vi "Check MCP Names.vi"(8 "error in":errorcluster, 9 "kind (Control)":string="Control", 10 "labels":string[](array[string]), 11 "MCP names":string[](array[string])) -> (0 "error out":errorcluster)   [LabVIEW 2020, in "MCP Server.lvlib"]
doc: "Checks MCP names generated by To MCP Name.vi before a tool or prompt is registered. Returns error 5010 when a name is empty, when it is longer than 64 characters, or when two different labels map to the same MCP name. The error message names the offending label(s) and the generated name. Passes an incoming error through unchanged."
uses:
  MCP Server.lvlib
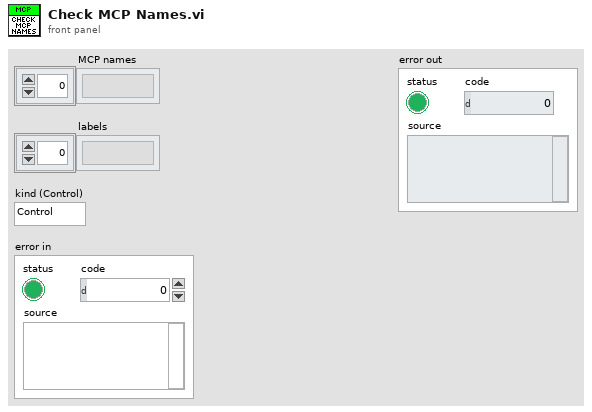
[diagram p1: front panel]
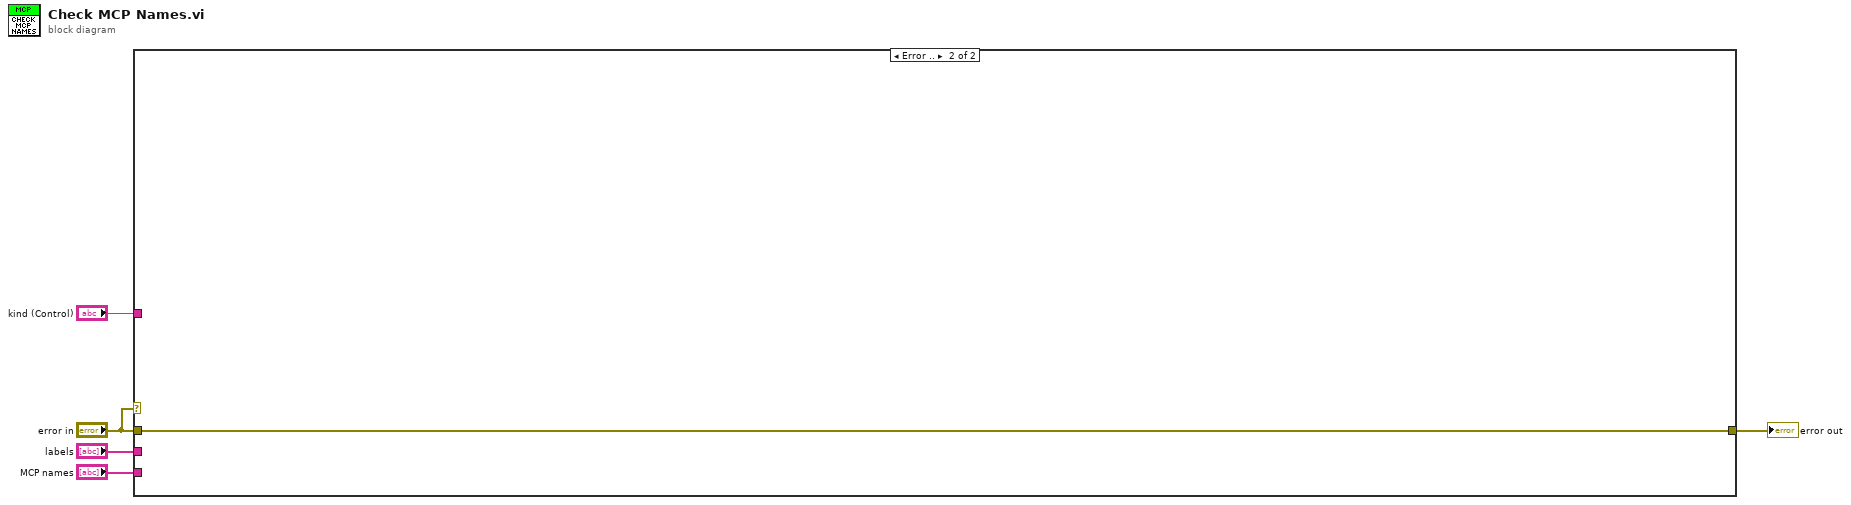
[diagram p0: block diagram]
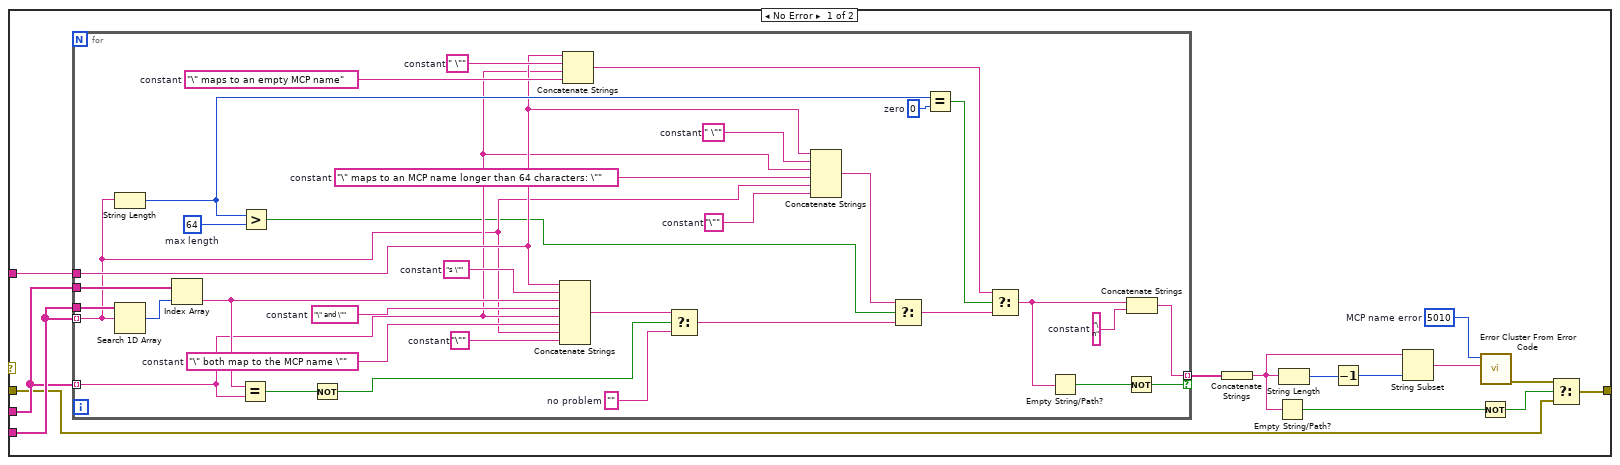
[diagram p2: hidden frame]
diagram:
  n1 = case shown="Error .." "error in" {
    tunnel: "MCP names" -> [w19 _]
    tunnel: "labels" -> [w18 _]
    tunnel: "kind (Control)" -> [w17 _]
    tunnel: "error in" -> [w7 w54]
    tunnel: [w6 w54] -> w1
    frame No Error {
      w11 = 5010  # MCP name error
      n2 = for {
        tunnel: w19 -> [w35] mode=indexing
        tunnel: w18 -> [w37] mode=indexing
        tunnel: w19 -> [w50]
        tunnel: w18 -> [w49]
        tunnel: w17 -> [w41]
        tunnel: [w20] -> w16 mode=indexing if=w21
        w22 = "\n"  # constant
        w31 = ""  # no problem
        w34 = "\""  # constant
        w36 = "\" both map to the MCP name \""  # constant
        w38 = "\" and \""  # constant
        w40 = "s \""  # constant
        w42 = "\""  # constant
        w43 = "\" maps to an MCP name longer than 64 characters: \""  # constant
        w44 = " \""  # constant
        w45 = "\" maps to an empty MCP name"  # constant
        w46 = " \""  # constant
        w51 = 64  # max length
        w53 = 0  # zero
        n3 = String Length(string=w35) -> (length=w52:i32)
        n4 = Search 1D Array(1D array=w50, element=w35) -> (index of element=w48:i32)  [unwired: 1 in]
        n5 = Index Array(array=w49, index=w48) -> (element=w39:string)
        n6 = Equal?(x=w39, y=w37) -> (x = y?=w47:bool)
        n7 = Greater?(x=w52, y=w51) -> (0:w29:bool)
        n8 = Not(x=w47) -> (.not. x?=w32:bool)
        n9 = Concatenate Strings(w41, w40, w39, w38, w37, w36, w35, w34) -> (w33:string)
        n10 = Concatenate Strings(w41, w46, w37, w45) -> (w27:string)
        n11 = Select(t=w33, s=w32, f=w31) -> (s? t:f=w28:string)
        n12 = Concatenate Strings(w41, w44, w37, w43, w35, w42) -> (w30:string)
        n13 = Select(t=w30, s=w29, f=w28) -> (s? t:f=w25:string)
        n14 = Equal?(x=w52, y=w53) -> (x = y?=w26:bool)
        n15 = Select(t=w27, s=w26, f=w25) -> (s? t:f=w23:string)
        n16 = Empty String/Path?(string/path=w23) -> (empty?=w24:bool)
        n17 = Not(x=w24) -> (.not. x?=w21:bool)
        n18 = Concatenate Strings(w23, w22) -> (w20:string)
      }
      n19 = Concatenate Strings(w16) -> (w13:string)
      n20 = Empty String/Path?(string/path=w13) -> (empty?=w12:bool)
      n21 = String Length(string=w13) -> (length=w15:i32)
      n22 = Decrement(x=w15) -> (x-1=w14:i32)
      n23 = String Subset(string=w13, length (rest)=w14) -> (substring=w10:string)  [unwired: 1 in]
      n24 = Not(x=w12) -> (.not. x?=w8:bool)
      n25 = call <vilib>:"Error Cluster From Error Code.vi"("error message (\"\")"=w10, "error code (0)"=w11) -> ("error out"=w9:errorcluster)  [unwired: 7 in]
      n26 = Select(t=w9, s=w8, f=w7) -> (s? t:f=w6:errorcluster)
    }
    frame Error {
    }
  }
  "error out" <- w1
